vi "VirtualATE_V2_after_step8.vi"() -> ()   [LabVIEW 2026]
uses:
  <vilib>/NI/Modbus Library/API/Modbus API.lvclass/Modbus API.ctl
  <vilib>/NI/Modbus Library/Transmission Data Unit/Transmission Data Unit.lvclass/Transmission Data Unit.ctl
  <vilib>/NI/Modbus Library/Transmission Data Unit/Write Unit ID.vi
  <vilib>/NI/Modbus Library/API/Read Transmission Data Unit.vi
  <vilib>/NI/Modbus Library/API/Write Transmission Data Unit.vi
  <vilib>/NI/Modbus Library/API/Master/Modbus Master.lvclass
  C:/Program Files (x86)/National Instruments/LabVIEW 2026/vi.lib/NI/Modbus Library/API/Modbus API.lvclass
  <vilib>/NI/Modbus Library/API/Wrapper/Create TCP Master.vi
  <vilib>/NI/Modbus Library/API/Wrapper/API Main.lvlib
panel:
  out "PLC_HB_TIMEOUT":bool
  out "PLC_HB_AGE_MS":u32
  out "PLC_LIVE_OK":bool
  out "STATE_ELAPSED_MS":u32
  out "처리 메시지":string
  out "ATE_READY":bool
  out "ACTIVE_RESULT":u16
  out "ACTIVE_ID":u16
  out "ATE_STATE":u16
  out "PLC_LIVE_COUNTER":u16
  out "PLC_ACCEPTED_ID":u16
  out "PLC_RX_RESPONSE_ID":u16
  out "PLC_RX_DONE":u16
  out "PLC_RX_RESULT":u16
  in  "검사 결과 선택":enum16{"PASS", "FAIL", "RETEST"}(ring)
  out "바깥 Tick Count(ms)":u32
  in  "ATE 읽기 정지":bool
  out "ALARM_CODE":u16
  out "SEQ_STATE":u16
  out "TEEST_RESULT_LATCH":u16
  out "ATE_DONE":u16
  out "ATE_RESPONSE_ID":u16
  out "ATE_RESULT":u16
  out "ATE_REQUEST_ID":u16
  out "ATE_REQUEST":u16
  out "마지막 Modbus 읽기 정상":bool
  out "수신 레지스터":u16[](array[numeric])
  out "error out":errorcluster
  in  "Unit ID":u8
  in  "Port":u16
  in  "Server IP":string
  # "R[3]"
  # "R[4]"
  # "R[5]"
  # "R[6]"
  # "R[7]"
  # "R[8]"
  # "R[9]"
  # "R[10]"
  # "R[11]"
  # "R[12]"
  # "0 ATE_LINK_TEST\n1 ATE_REQUEST\n2 ATE_REQUEST_ID\n3 ATE_RESULT\n4 ATE_RESPONSE_ID\n5 ATE_DONE\n6 TEST_RESULT_LATCH\n7 SEQ_STATE\n8 ALARM_CODE"
  # "R[13]"
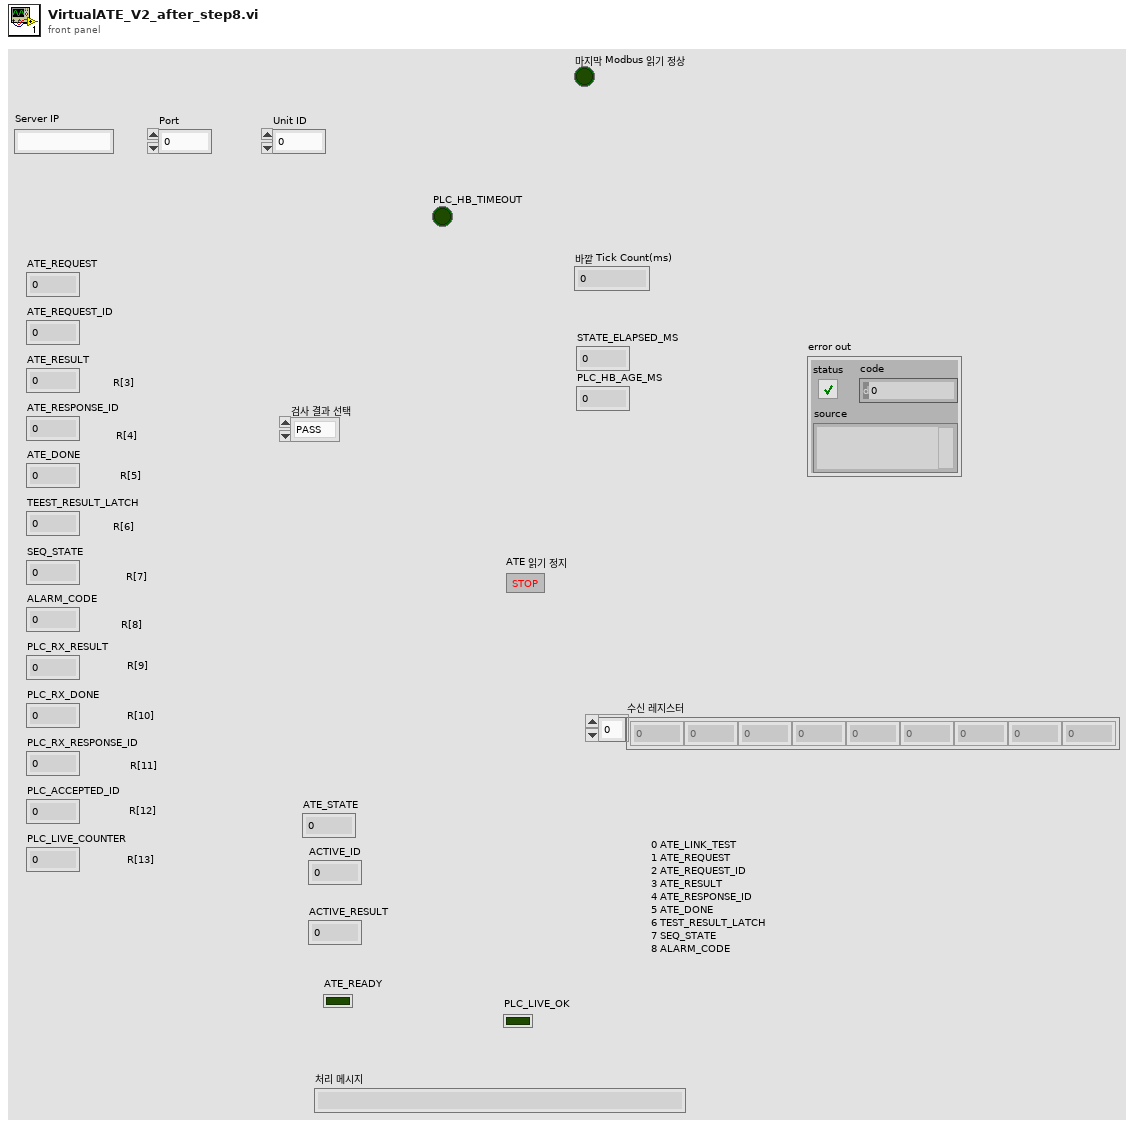
[diagram p1: front panel]
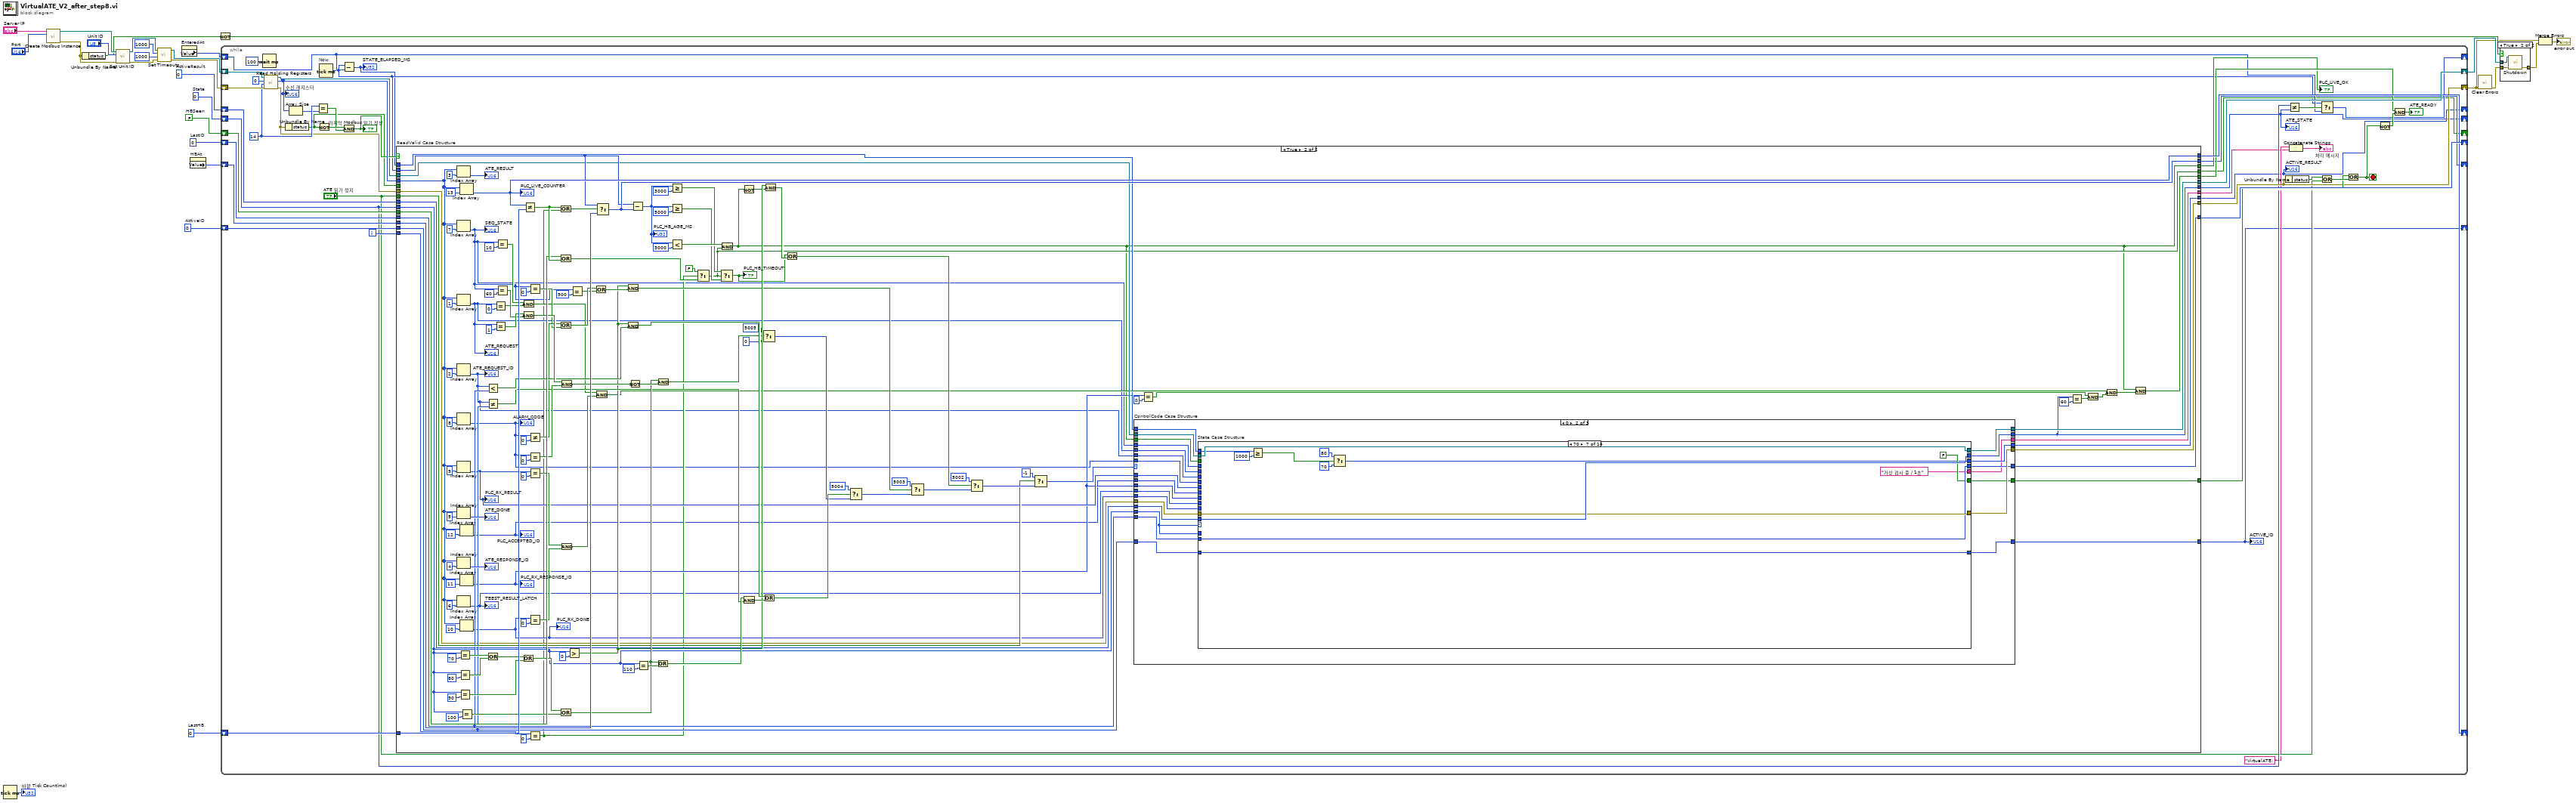
[diagram p0: block diagram]
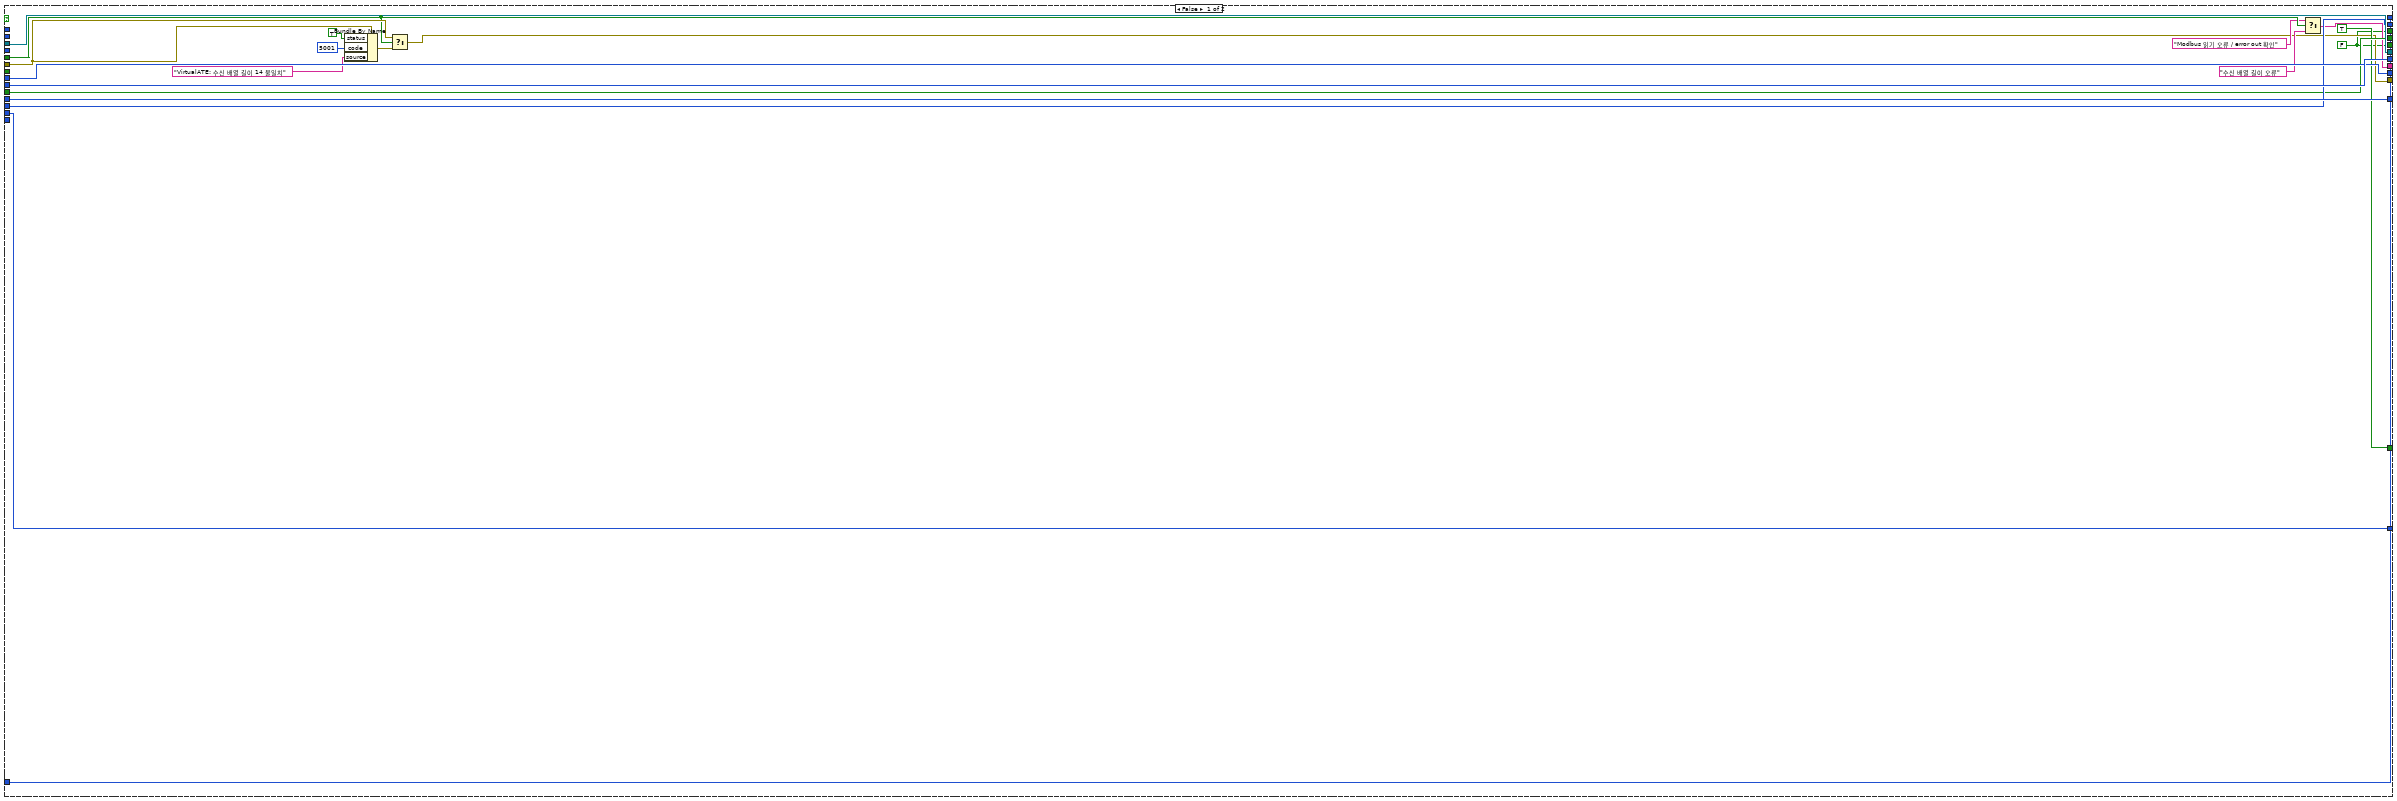
[diagram p3: hidden frame]
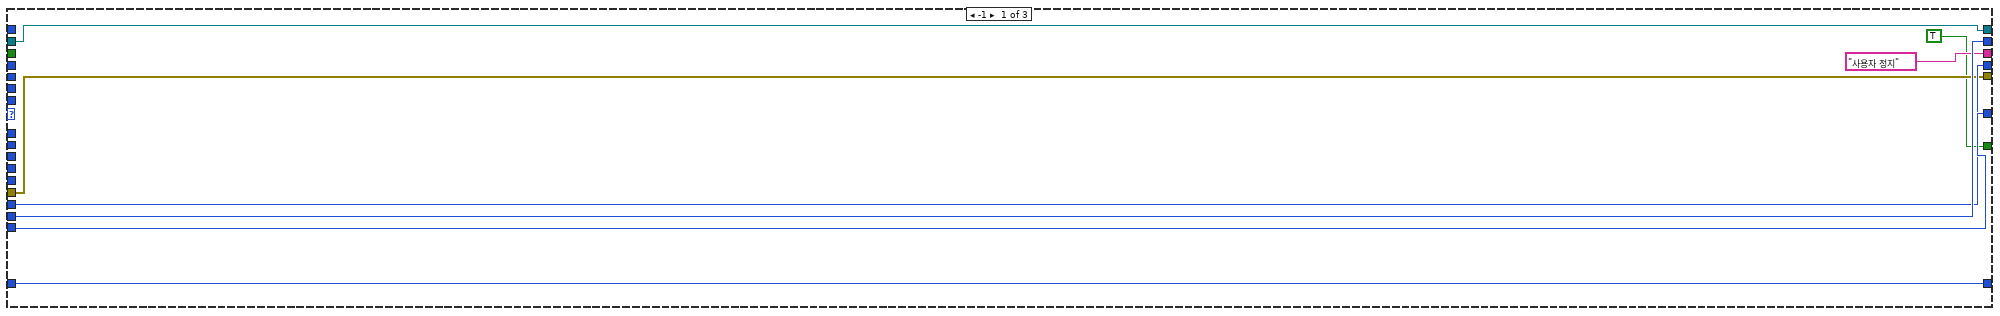
[diagram p4: hidden frame]
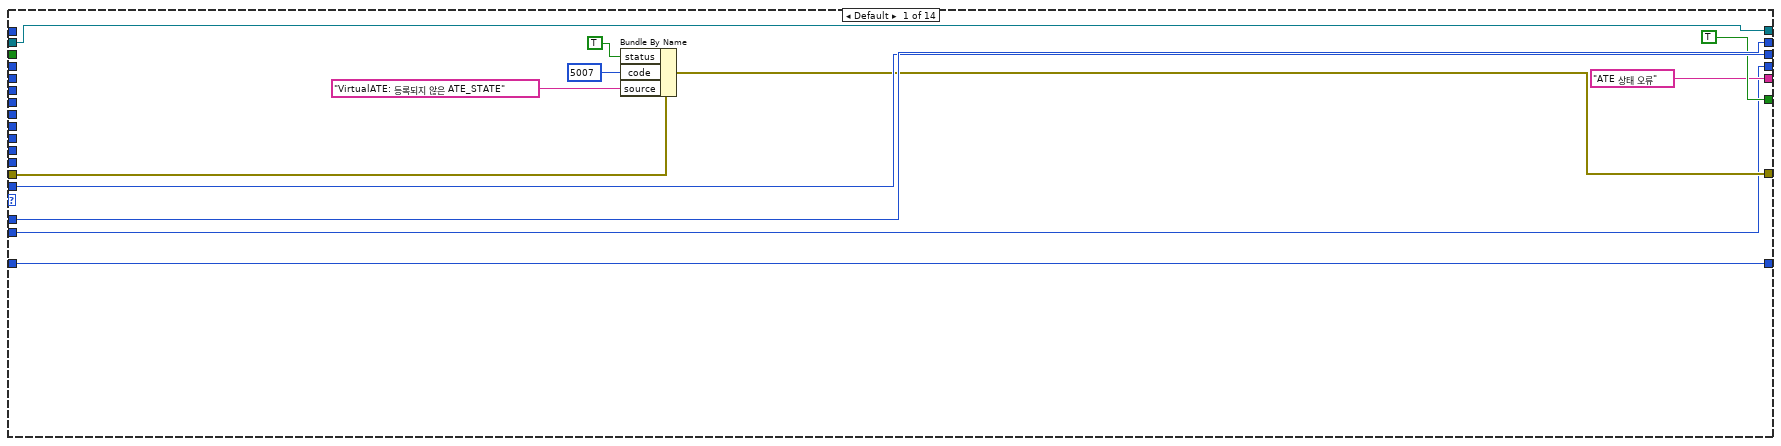
[diagram p5: hidden frame]
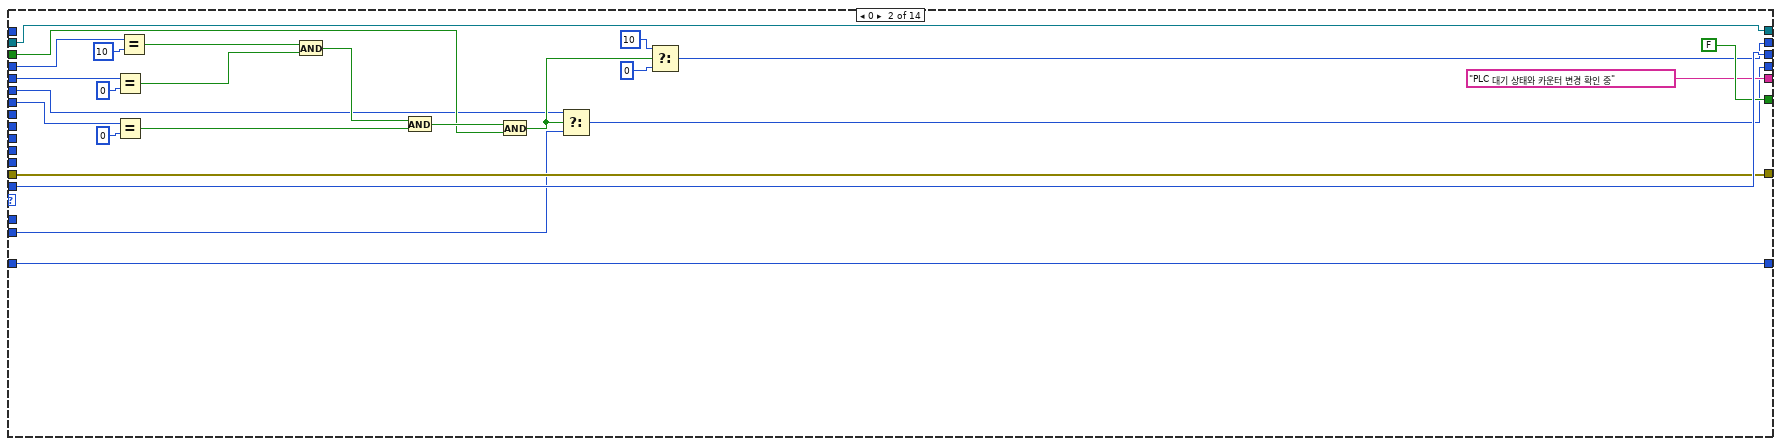
[diagram p6: hidden frame]
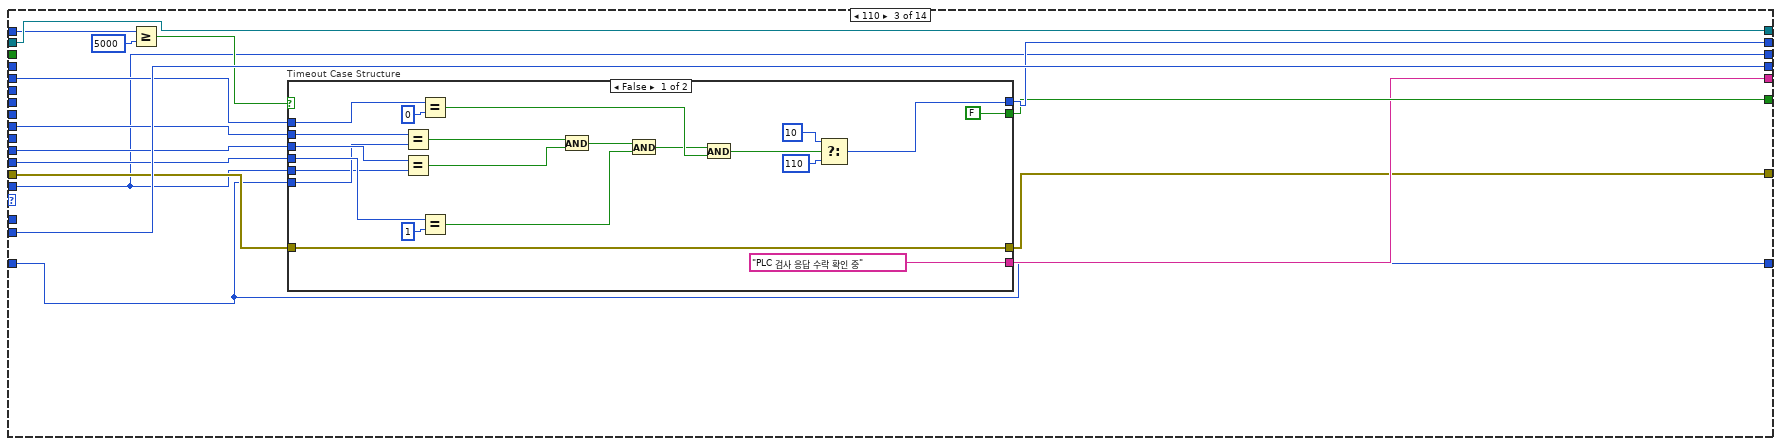
[diagram p7: hidden frame]
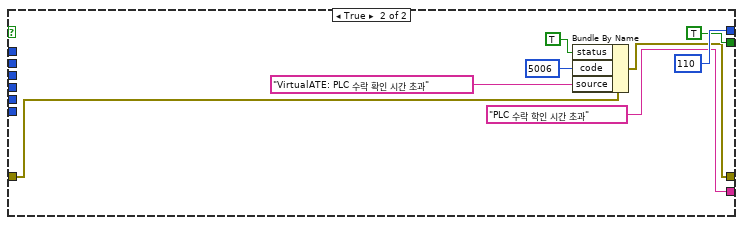
[diagram p8: hidden frame]
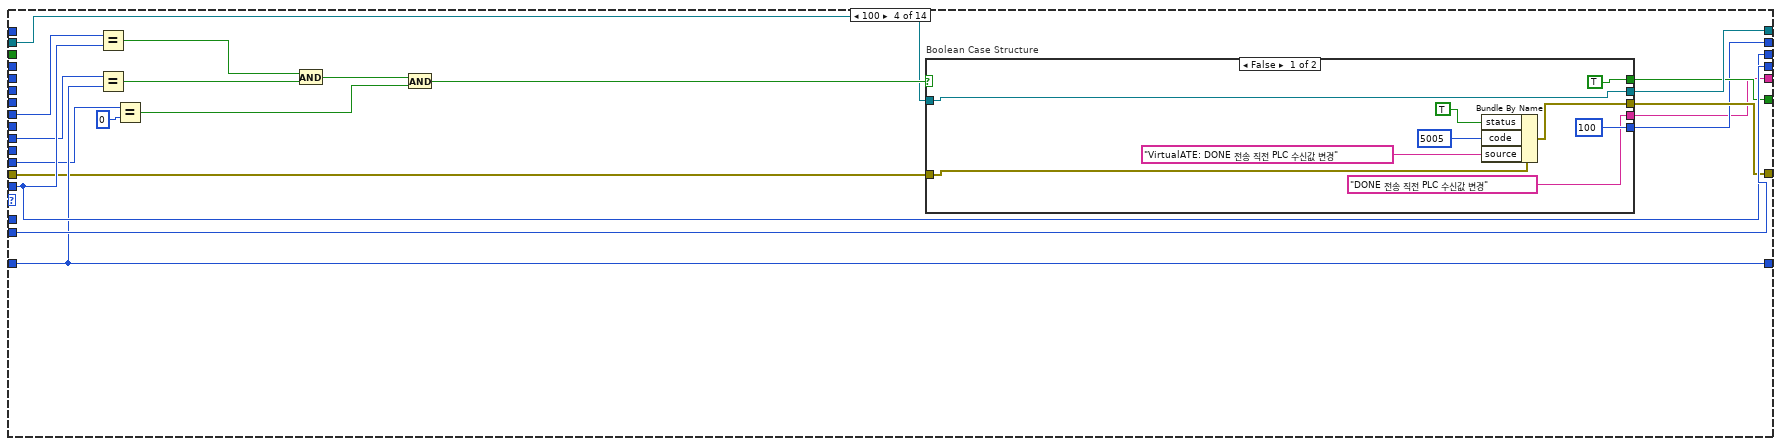
[diagram p9: hidden frame]
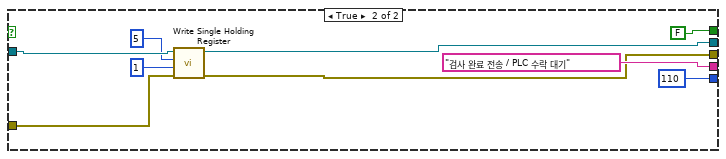
[diagram p10: hidden frame]
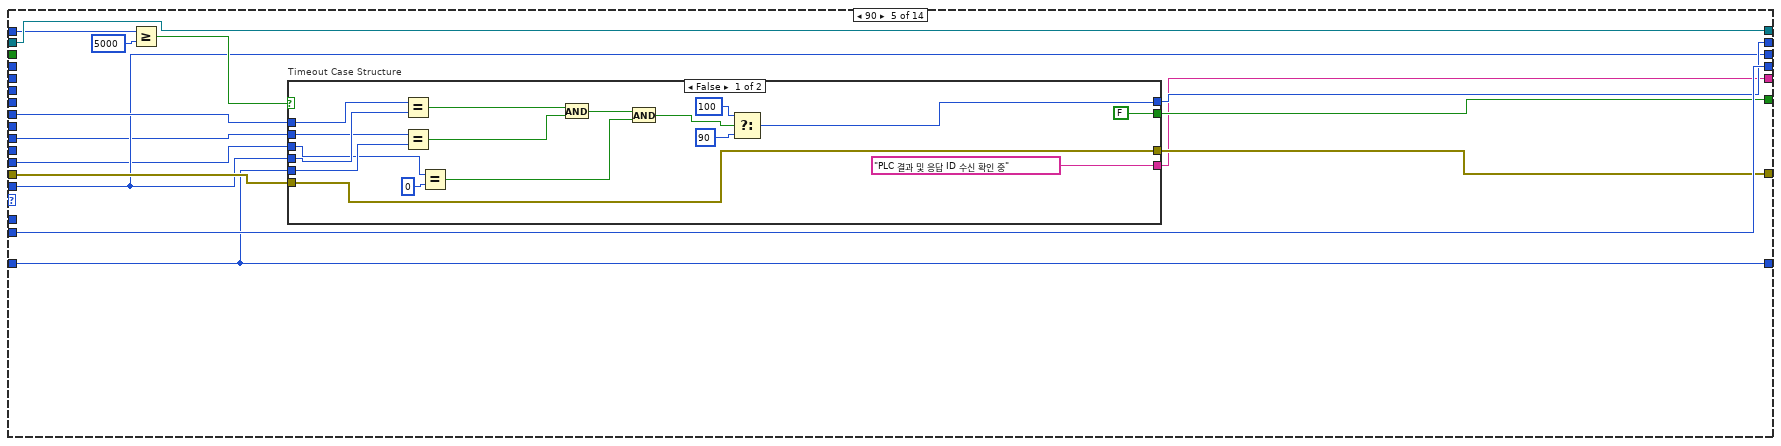
[diagram p11: hidden frame]
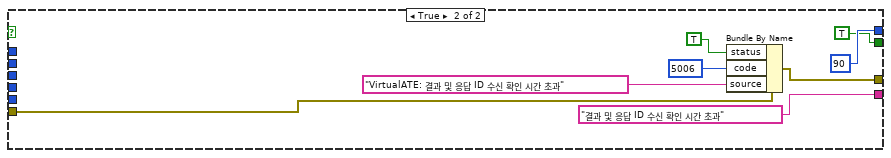
[diagram p12: hidden frame]
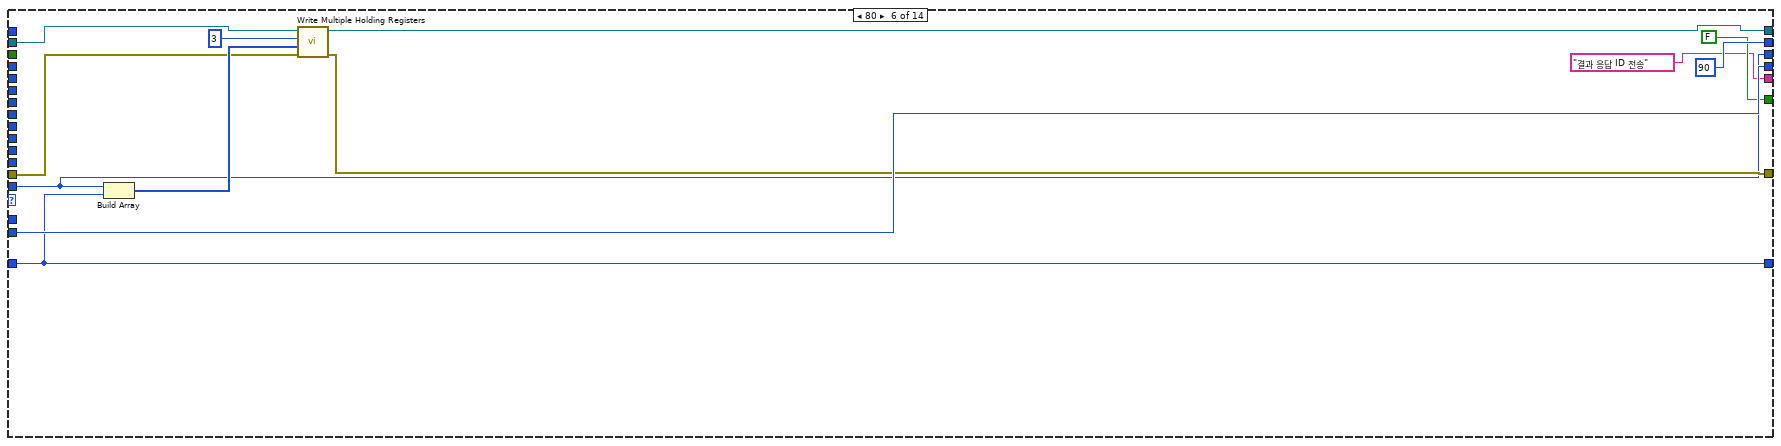
[diagram p13: hidden frame]
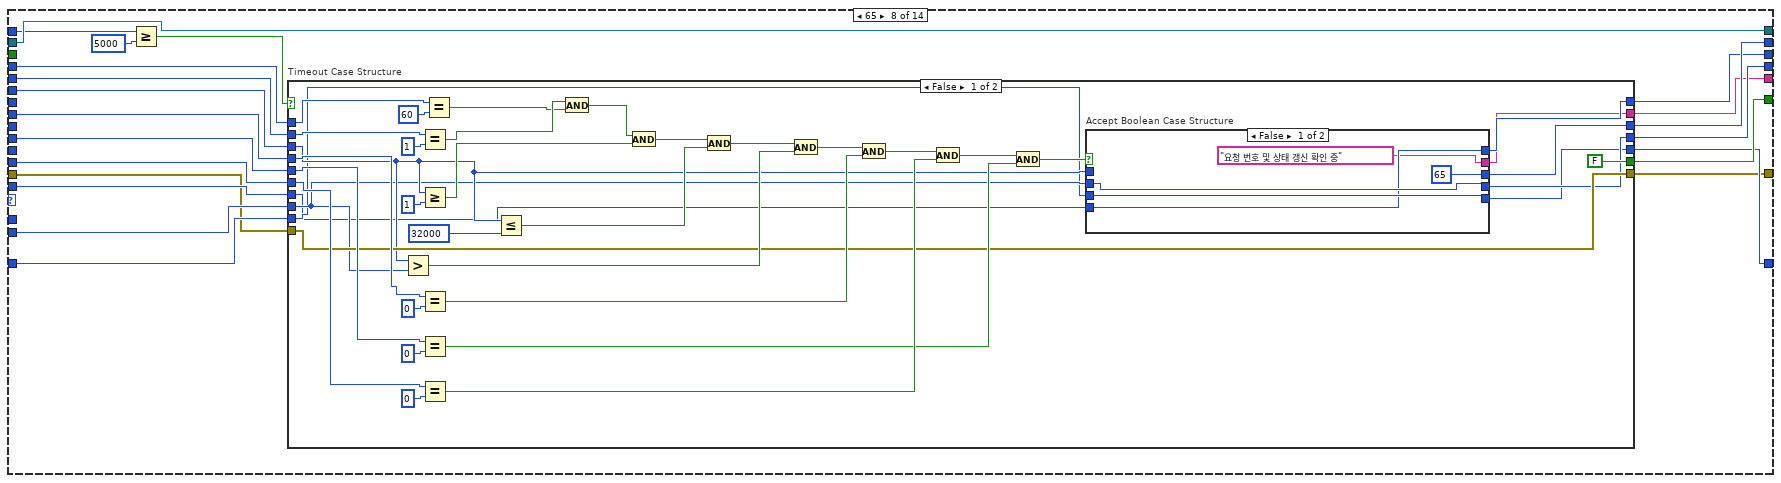
[diagram p14: hidden frame]
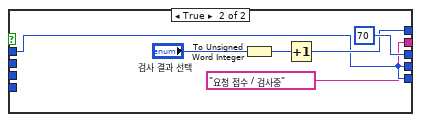
[diagram p15: hidden frame]
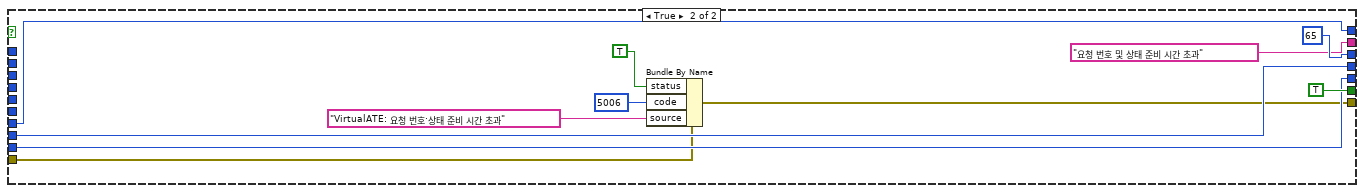
[diagram p16: hidden frame]
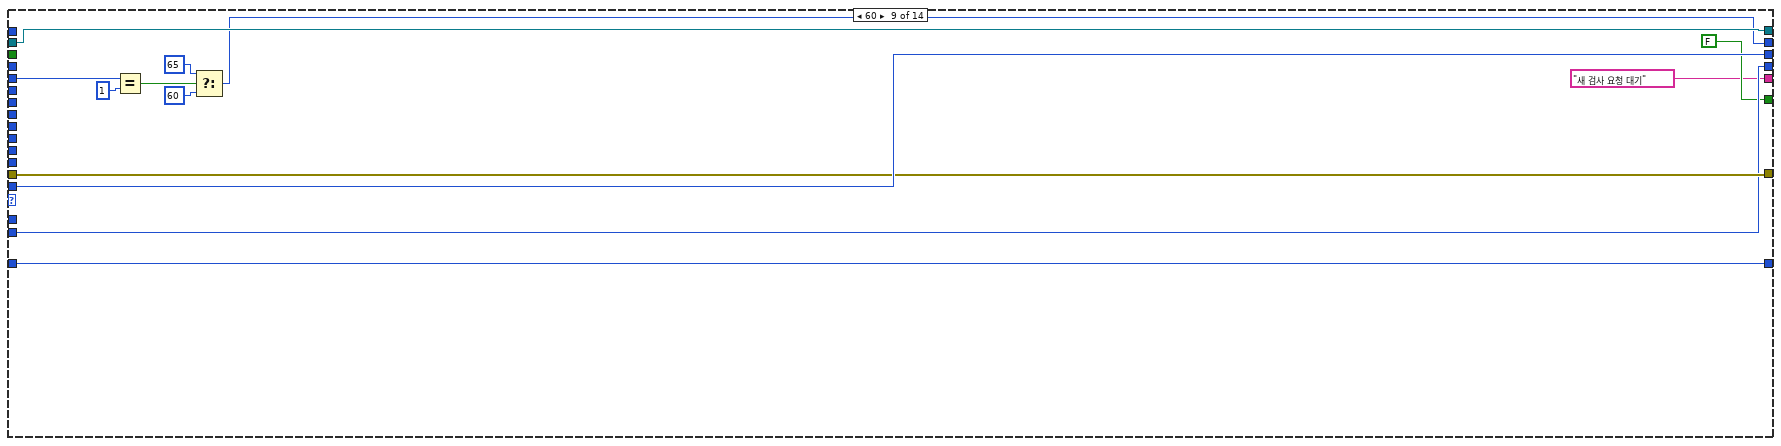
[diagram p17: hidden frame]
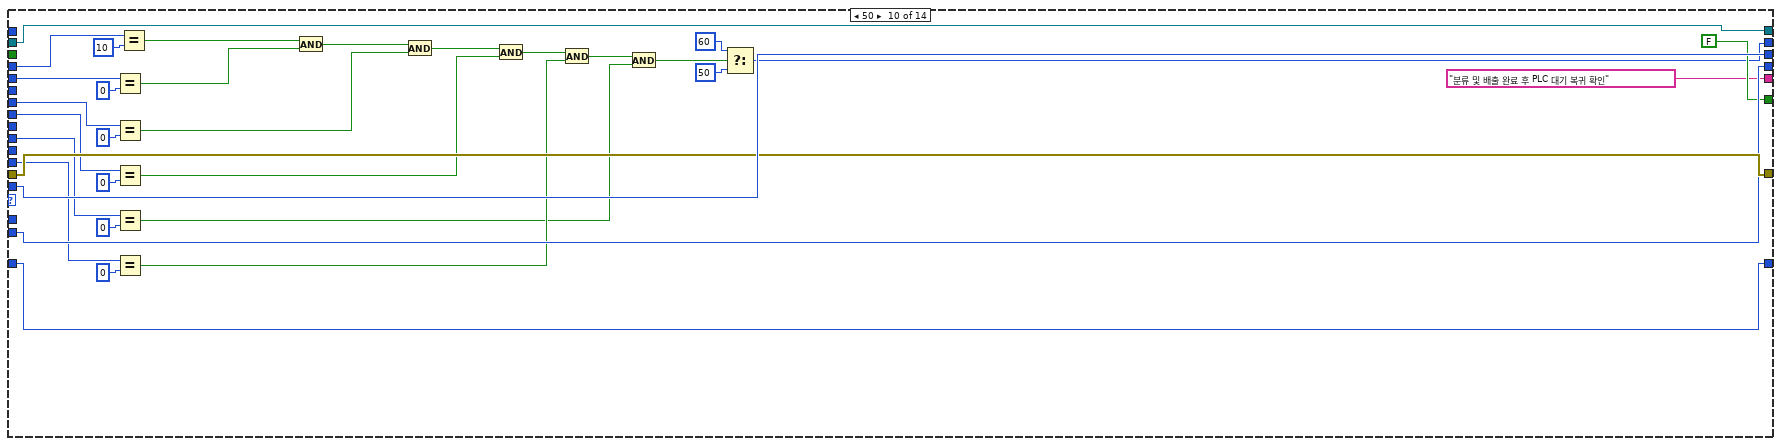
[diagram p18: hidden frame]
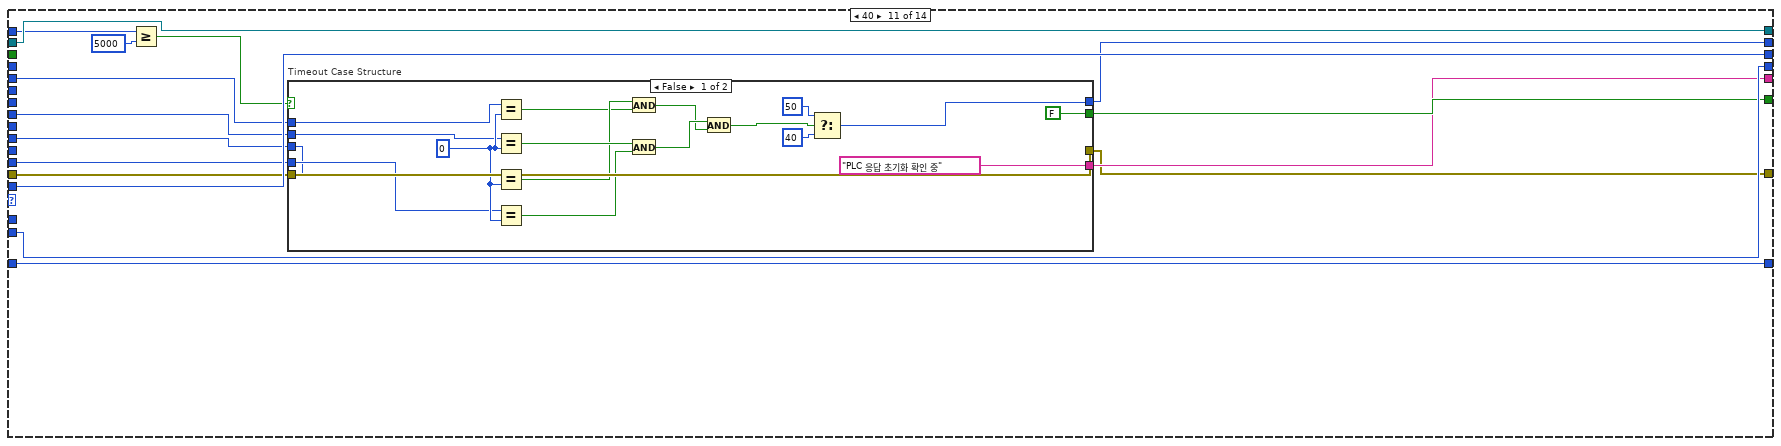
[diagram p19: hidden frame]
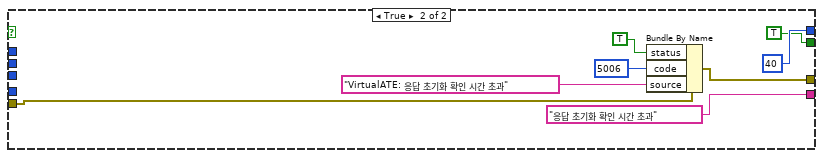
[diagram p20: hidden frame]
diagram:
  w9 = FALSE  # HBSeen
  w4 = u16 0  # LastHB
  w5 = u16 0  # ActiveResult
  w6 = u16 0  # ActiveID
  w7 = u16 0  # LastID
  w8 = u16 0  # State
  n1 = Tick Count (ms)() -> (millisecond timer value=→"바깥 Tick Count(ms)":u32)
  n2 = call-poly <vilib>:"Create Modbus Instance.vi"("port (502)"="Port", "address"="Server IP") -> ("error out"=w17:errorcluster, "TCP master instance"=w22:refnum<class "Modbus Master.lvclass">)  [unwired: 8 in]
  n3 = Unbundle By Name(w17) -> ("status"=w16:bool)
  n4 = call <vilib>:"Set Unit ID.vi"("error in"=w17, "unit ID"="Unit ID", "Modbus master in"=w22) -> ("error out"=w20:errorcluster, "Modbus master out"=w21:refnum<class "Modbus Master.lvclass">)  [unwired: 7 in]
  n5 = call <vilib>:"Set Timeouts.vi"("error in"=w20, "write operation timeout"=1000, "read operation timeout"=1000, "Modbus master in"=w21) -> ("error out"=w18:errorcluster, "Modbus master out"=w19:refnum<class "Modbus Master.lvclass">)  [unwired: 6 in]
  n6 = property on="EnteredAt" class="DigNum (strict)"() -> ("Value"=w2:u32)  [unwired: 2 in, 2 out]
  n7 = property on="HBAt" class="DigNum (strict)"() -> ("Value"=w1:u32)  [unwired: 2 in, 2 out]
  n8 = Not(x=w16) -> (.not. x?=w15:bool)
  n9 = while {
    shift-right: [w48] -> w11
    shift-left: w18 -> [w71]
    shift-right: [w59] -> w14
    shift-left: w19 -> [w72]
    shift-right: [w28] -> _
    shift-left: w8 -> [w40]
    shift-right: [w63] -> _
    shift-left: w7 -> [w64]
    shift-right: [w30] -> _
    shift-left: w6 -> [w62]
    shift-right: [w29] -> _
    shift-left: w5 -> [w61]
    shift-right: [w38] -> _
    shift-left: w1 -> [w55]
    shift-right: [w56] -> _
    shift-left: w4 -> [w57]
    shift-right: [w42] -> _
    shift-left: w2 -> [w39]
    shift-right: [w37] -> _
    shift-left: w9 -> [w54]
    i -> [w43]
    stop <- w45 stop-if-true
    w70 = u16 14 ("number of inputs")
    n10 = Wait (ms)(milliseconds to wait=u32 100) -> ()  [unwired: 1 out]
    n11 = call-dynamic "Read Holding Registers.vi"("error in"=w71, "number of inputs"=w70, "starting address"=u16 0, "Modbus master in"=w72) -> ("error out"=w58:errorcluster, "register values"=w66:u16[], "Modbus master out"=w60:refnum<class "Modbus Master.lvclass">)  [unwired: 5 in]
    "수신 레지스터" <- w66
    n12 = Unbundle By Name(w58) -> ("status"=w53:bool)
    n13 = Array Size(array=w66) -> (size(s)=w69:i32)
    n14 = Equal?(x=w70, y=w69) -> (x = y?=w67:bool)
    n15 = Not(x=w53) -> (.not. x?=w68:bool)
    n16 = Tick Count (ms) "Now"() -> (millisecond timer value=w36:u32)
    n17 = Subtract(x=w36, y=w39) -> (x-y=w34:u32)
    "STATE_ELAPSED_MS" <- w34
    n18 = And(x=w68, y=w67) -> (x .and. y?=w65:bool)
    "마지막 Modbus 읽기 정상" <- w65
    n19 = case "ReadValid Case Structure" shown="True" w65 {
      tunnel: w66 -> [_ w220]
      tunnel: w40 -> [w94 w127]
      tunnel: [w94 w121] -> w28
      tunnel: w64 -> [w93 w139]
      tunnel: [w93 w138] -> w63
      tunnel: w62 -> [w92 w137]
      tunnel: [w92 w136] -> w30
      tunnel: w61 -> [w91 w135]
      tunnel: [w91 w134] -> w29
      tunnel: w60 -> [w90 w133]
      tunnel: [w90 w132] -> w59
      tunnel: w58 -> [w82 w131]
      tunnel: [w76 w130] -> w48
      tunnel: w57 -> [w89 w212]
      tunnel: [w89 w209] -> w56
      tunnel: w55 -> [w88 w207]
      tunnel: [w88 w208] -> w38
      tunnel: w54 -> [w87 w210]
      tunnel: [w87 w102] -> w37
      tunnel: w53 -> [w80 _]
      tunnel: [TRUE w128] -> w51
      tunnel: [w77 w129] -> w32
      tunnel: [w75 w108] -> w49
      tunnel: [w75 w95] -> w44
      tunnel: w43 -> [_ w214]
      tunnel: w36 -> [_ w201]
      tunnel: "ATE 읽기 정지" -> [_ w141]
      tunnel: w34 -> [_ w107]
      frame False {
        w75 = FALSE
        n20 = Bundle By Name(cluster=w82, "status"=TRUE, "code"=5001, "source"="VirtualATE: 수신 배열 길이 14 불일치") -> (w83:errorcluster)
        n21 = Select(t=w82, s=w80, f=w83) -> (s? t:f=w76:errorcluster)
        n22 = Select(t="Modbus 읽기 오류 / error out 확인", s=w80, f="수신 배열 길이 오류") -> (s? t:f=w77:string)
      }
      frame True {
        n23 = Index Array(array=w220, index=3) -> (element=→"ATE_RESULT":u16)
        n24 = Index Array(array=w220, index=7) -> (element=w100:u16)
        "SEQ_STATE" <- w100
        n25 = Index Array(array=w220, index=1) -> (element=w103:u16)
        "ATE_REQUEST" <- w103
        n26 = Index Array(array=w220, index=2) -> (element=w98:u16)
        "ATE_REQUEST_ID" <- w98
        n27 = Index Array(array=w220, index=8) -> (element=w99:u16)
        "ALARM_CODE" <- w99
        n28 = Index Array(array=w220, index=9) -> (element=w105:u16)
        "PLC_RX_RESULT" <- w105
        n29 = Index Array(array=w220, index=5) -> (element=→"ATE_DONE":u16)
        n30 = Index Array(array=w220, index=4) -> (element=→"ATE_RESPONSE_ID":u16)
        n31 = Index Array(array=w220, index=6) -> (element=w96:u16)
        "TEEST_RESULT_LATCH" <- w96
        n32 = Equal?(x=w127, y=u16 70) -> (x = y?=w190:bool)
        n33 = Equal?(x=w127, y=u16 80) -> (x = y?=w189:bool)
        n34 = Equal?(x=w127, y=u16 90) -> (x = y?=w188:bool)
        n35 = Index Array(array=w220, index=13) -> (element=w209:u16)
        "PLC_LIVE_COUNTER" <- w209
        n36 = Index Array(array=w220, index=12) -> (element=w97:u16)
        "PLC_ACCEPTED_ID" <- w97
        n37 = Index Array(array=w220, index=11) -> (element=w104:u16)
        "PLC_RX_RESPONSE_ID" <- w104
        n38 = Index Array(array=w220, index=10) -> (element=w106:u16)
        "PLC_RX_DONE" <- w106
        n39 = Equal?(x=w127, y=u16 100) -> (x = y?=w186:bool)
        n40 = Less?(x=w98, y=w139) -> (x < y?=w172:bool)
        n41 = Not Equal?(x=w98, y=w137) -> (x != y?=w170:bool)
        n42 = Or(x=w190, y=w189) -> (x .or. y?=w187:bool)
        n43 = Equal?(x=w103, y=u16 0) -> (x = y?=w118:bool)
        n44 = Equal?(x=w103, y=u16 1) -> (x = y?=w179:bool)
        n45 = Equal?(x=w100, y=u16 10) -> (x = y?=w119:bool)
        n46 = Equal?(x=w100, y=u16 60) -> (x = y?=w178:bool)
        n47 = Or(x=w187, y=w188) -> (x .or. y?=w185:bool)
        n48 = And(x=w119, y=w118) -> (x .and. y?=w113:bool)
        n49 = And(x=w179, y=w178) -> (x .and. y?=w176:bool)
        n50 = Not Equal?(x=w209, y=w212) -> (x != y?=w211:bool)
        n51 = Equal?(x=w100, y=u16 0) -> (x = y?=w163:bool)
        n52 = Not Equal?(x=w99, y=u16 0) -> (x != y?=w164:bool)
        n53 = Equal?(x=w99, y=u16 0) -> (x = y?=w177:bool)
        n54 = Equal?(x=w105, y=u16 0) -> (x = y?=w117:bool)
        n55 = Equal?(x=w106, y=u16 0) -> (x = y?=w116:bool)
        n56 = Equal?(x=w214, y=0) -> (x = y?=w101:bool)
        n57 = Or(x=w211, y=w101) -> (x .or. y?=w205:bool)
        n58 = Or(x=w210, y=w211) -> (x .or. y?=w206:bool)
        n59 = Or(x=w164, y=w163) -> (x .or. y?=w162:bool)
        n60 = Or(x=w185, y=w186) -> (x .or. y?=w173:bool)
        n61 = And(x=w176, y=w177) -> (x .and. y?=w175:bool)
        n62 = And(x=w117, y=w116) -> (x .and. y?=w112:bool)
        n63 = Greater?(x=w127, y=u16 0) -> (0:w159:bool)
        n64 = Equal?(x=w100, y=u16 900) -> (x = y?=w161:bool)
        n65 = Or(x=w162, y=w161) -> (x .or. y?=w160:bool)
        n66 = And(x=w113, y=w112) -> (x .and. y?=w110:bool)
        n67 = Select(t=w201, s=w205, f=w207) -> (s? t:f=w208:u32)
        n68 = And(x=w159, y=w160) -> (x .and. y?=w151:bool)
        n69 = And(x=w159, y=w172) -> (x .and. y?=w169:bool)
        n70 = Not(x=w175) -> (.not. x?=w174:bool)
        n71 = Subtract(x=w201, y=w208) -> (x-y=w200:u32)
        "PLC_HB_AGE_MS" <- w200
        n72 = Equal?(x=w127, y=u16 110) -> (x = y?=w183:bool)
        n73 = Or(x=w173, y=w183) -> (x .or. y?=w171:bool)
        n74 = And(x=w173, y=w174) -> (x .and. y?=w155:bool)
        n75 = Greater Or Equal?(x=w200, y=u32 3000) -> (x >= y?=w197:bool)
        n76 = Greater Or Equal?(x=w200, y=u32 5000) -> (x >= y?=w196:bool)
        n77 = Less?(x=w200, y=u32 3000) -> (x < y?=w203:bool)
        n78 = Select(t=FALSE, s=w101, f=w206) -> (s? t:f=w102:bool)
        n79 = Select(t=w197, s=w102, f=w196) -> (s? t:f=w156:bool)
        "PLC_HB_TIMEOUT" <- w156
        n80 = And(x=w203, y=w102) -> (x .and. y?=w95:bool)
        n81 = Not(x=w95) -> (.not. x?=w158:bool)
        n82 = And(x=w171, y=w170) -> (x .and. y?=w168:bool)
        n83 = Select(t=5005, s=w155, f=0) -> (s? t:f=w148:i32)
        n84 = Or(x=w169, y=w168) -> (x .or. y?=w152:bool)
        n85 = And(x=w159, y=w158) -> (x .and. y?=w157:bool)
        n86 = Or(x=w156, y=w157) -> (x .or. y?=w150:bool)
        n87 = Select(t=5004, s=w152, f=w148) -> (s? t:f=w147:i32)
        n88 = Select(t=5003, s=w151, f=w147) -> (s? t:f=w145:i32)
        n89 = Select(t=5002, s=w150, f=w145) -> (s? t:f=w143:i32)
        n90 = Select(t=-1, s=w141, f=w143) -> (s? t:f=w140:i32)
        n91 = case "ControlCode Case Structure" shown="0" w140 {
          selector: w140 -> [_ _ w692]
          tunnel: w127 -> [w239 w247 w700]
          tunnel: [w239 w258 w700] -> w121
          tunnel: w139 -> [w238 w264 w699]
          tunnel: [w238 w255 w699] -> w138
          tunnel: w137 -> [w237 w263 w698]
          tunnel: [w237 w254 w698] -> w136
          tunnel: [w236 w260 w697] -> w134
          tunnel: w135 -> [w236 w262 w697]
          tunnel: [w235 w259 w696] -> w132
          tunnel: w133 -> [w235 w261 w696]
          tunnel: [w234 w257 w695] -> w130
          tunnel: w131 -> [w234 w256 w694]
          tunnel: ["사용자 정지" w252 w674] -> w129
          tunnel: [TRUE w253 TRUE] -> w128
          tunnel: w107 -> [_ w251 _]
          tunnel: w106 -> [_ w250 _]
          tunnel: w105 -> [_ w249 _]
          tunnel: w104 -> [_ w248 _]
          tunnel: w103 -> [_ w244 _]
          tunnel: w100 -> [_ w246 _]
          tunnel: w99 -> [_ w245 _]
          tunnel: w98 -> [_ w243 _]
          tunnel: w97 -> [_ w242 _]
          tunnel: w96 -> [_ w241 _]
          tunnel: w95 -> [_ w240 _]
          frame -1 {
          }
          frame 0 {
            n92 = case "State Case Structure" shown="70" w247 {
              tunnel: w264 -> [w265 w278 w316 w365 w397 w434 w445 w464 w539 w572 w589 w629 w642 w671]
              tunnel: w263 -> [w266 w298 w303 w361 w385 w424 w444 w460 w538 w571 w588 w628 w641 w670]
              tunnel: w262 -> [w275 w301 w302 w363 w387 w425 w448 w458 w542 w575 w591 w631 w644 w673]
              tunnel: w261 -> [w274 w300 w317 w351 w398 w428 w447 w469 w541 w574 w590 w625 w643 w667]
              tunnel: [w275 w301 w302 w363 w387 w425 w448 w457 w542 w575 w591 w631 w644 w673] -> w260
              tunnel: [w274 w300 w317 w350 w398 w426 w447 w469 w541 w574 w590 w623 w643 w666] -> w259
              tunnel: [w276 w280 w312 w348 w391 u16 90 w439 w465 w530 w545 w582 u16 40 w635 u16 20] -> w258
              tunnel: [w269 w299 w308 w352 w392 w427 w446 w455 w540 w573 w580 w622 w634 w665] -> w257
              tunnel: w256 -> [w273 w299 w309 w353 w393 w429 w446 w456 w540 w573 w581 w624 w633 w664]
              tunnel: [w265 w277 w316 w365 w397 w434 w445 w463 w539 w572 w589 w629 w642 w671] -> w255
              tunnel: [w266 w298 w303 w361 w385 w424 w444 w459 w538 w571 w588 w628 w641 w670] -> w254
              tunnel: [TRUE FALSE w311 w349 w390 FALSE FALSE w462 FALSE FALSE w584 FALSE w636 FALSE] -> w253
              tunnel: ["ATE 상태 오류" "PLC 대기 상태와 카운터 변경 확인 중" w310 w347 w389 "결과 응답 ID 전송" "가상 검사 중 / 1초" w461 "새 검사 요청 대기" "분류 및 배출 완료 후 PLC 대기 복귀 확인" w583 "결과 및 응답 ID 초기화 전송" w637 "DONE=0 전송 / PLC 반영 대기"] -> w252
              tunnel: w247 -> [w276 _ _ _ _ _ _ _ _ _ _ _ _ _]
              tunnel: w251 -> [_ _ w315 _ w396 _ w437 w467 _ _ w586 _ w639 _]
              tunnel: w250 -> [_ _ w305 w360 w384 _ _ w450 _ w564 w578 _ w632 _]
              tunnel: w249 -> [_ _ _ w364 w388 _ _ w451 _ w565 w579 _ _ _]
              tunnel: w248 -> [_ _ _ w362 w386 _ _ w449 _ w563 w577 _ _ _]
              tunnel: w244 -> [_ w293 w304 _ _ _ _ w454 w535 w567 w576 _ _ _]
              tunnel: w246 -> [_ w295 _ _ _ _ _ w453 _ w568 _ _ _ _]
              tunnel: w245 -> [_ w292 _ _ _ _ _ _ _ w566 _ _ _ _]
              tunnel: w243 -> [_ w279 _ _ _ _ _ w452 _ _ _ _ _ _]
              tunnel: w242 -> [_ _ w307 _ _ _ _ _ _ _ _ _ _ _]
              tunnel: w241 -> [_ _ w306 _ _ _ _ _ _ _ _ _ _ _]
              tunnel: w240 -> [_ w284 _ _ _ _ _ _ _ _ _ _ _ _]
              frame Default {
                n93 = Bundle By Name(cluster=w273, "status"=TRUE, "code"=5007, "source"="VirtualATE: 등록되지 않은 ATE_STATE") -> (w269:errorcluster)
              }
              frame 0 {
                n94 = Equal?(x=w293, y=u16 0) -> (x = y?=w288:bool)
                n95 = Equal?(x=w292, y=u16 0) -> (x = y?=w287:bool)
                n96 = Equal?(x=w295, y=u16 10) -> (x = y?=w289:bool)
                n97 = And(x=w289, y=w288) -> (x .and. y?=w286:bool)
                n98 = And(x=w286, y=w287) -> (x .and. y?=w285:bool)
                n99 = And(x=w285, y=w284) -> (x .and. y?=w283:bool)
                n100 = Select(t=w279, s=w283, f=w278) -> (s? t:f=w277:u16)
                n101 = Select(t=u16 10, s=w283, f=u16 0) -> (s? t:f=w280:u16)
              }
              frame 110 {
                n102 = Greater Or Equal?(x=w315, y=u32 5000) -> (x >= y?=w313:bool)
                n103 = case "Timeout Case Structure" shown="False" w313 {
                  tunnel: [w318 u16 110] -> w312
                  tunnel: [FALSE TRUE] -> w311
                  tunnel: ["PLC 검사 응답 수락 확인 중" "PLC 수락 학인 시간 초과"] -> w310
                  tunnel: w309 -> [w336 w343]
                  tunnel: [w336 w339] -> w308
                  tunnel: w307 -> [w335 _]
                  tunnel: w306 -> [w334 _]
                  tunnel: w305 -> [w333 _]
                  tunnel: w304 -> [w332 _]
                  tunnel: w303 -> [w331 _]
                  tunnel: w302 -> [w330 _]
                  frame False {
                    n104 = Equal?(x=w335, y=w331) -> (x = y?=w327:bool)
                    n105 = Equal?(x=w334, y=w330) -> (x = y?=w326:bool)
                    n106 = Equal?(x=w332, y=u16 0) -> (x = y?=w324:bool)
                    n107 = Equal?(x=w333, y=u16 1) -> (x = y?=w325:bool)
                    n108 = And(x=w327, y=w326) -> (x .and. y?=w323:bool)
                    n109 = And(x=w323, y=w325) -> (x .and. y?=w322:bool)
                    n110 = And(x=w322, y=w324) -> (x .and. y?=w321:bool)
                    n111 = Select(t=u16 10, s=w321, f=u16 110) -> (s? t:f=w318:u16)
                  }
                  frame True {
                    n112 = Bundle By Name(cluster=w343, "status"=TRUE, "code"=5006, "source"="VirtualATE: PLC 수락 확인 시간 초과") -> (w339:errorcluster)
                  }
                }
              }
              frame 100 {
                n113 = Equal?(x=w364, y=w363) -> (x = y?=w358:bool)
                n114 = Equal?(x=w362, y=w361) -> (x = y?=w357:bool)
                n115 = Equal?(x=w360, y=u16 0) -> (x = y?=w356:bool)
                n116 = And(x=w358, y=w357) -> (x .and. y?=w355:bool)
                n117 = And(x=w355, y=w356) -> (x .and. y?=w354:bool)
                n118 = case "Boolean Case Structure" shown="False" w354 {
                  tunnel: w353 -> [w370 w378]
                  tunnel: [w366 w377] -> w352
                  tunnel: w351 -> [w373 w380]
                  tunnel: [w373 w379] -> w350
                  tunnel: [TRUE FALSE] -> w349
                  tunnel: [u16 100 u16 110] -> w348
                  tunnel: ["DONE 전송 직전 PLC 수신값 변경" "검사 완료 전송 / PLC 수락 대기"] -> w347
                  frame False {
                    n119 = Bundle By Name(cluster=w370, "status"=TRUE, "code"=5005, "source"="VirtualATE: DONE 전송 직전 PLC 수신값 변경") -> (w366:errorcluster)
                  }
                  frame True {
                    n120 = call-dynamic "Write Single Holding Register.vi"("error in"=w378, "register to write"=u16 1, "address"=u16 5, "Modbus master in"=w380) -> ("error out"=w377:errorcluster, "Modbus master out"=w379:refnum<class "Modbus Master.lvclass">)  [unwired: 6 in]
                  }
                }
              }
              frame 90 {
                n121 = Greater Or Equal?(x=w396, y=u32 5000) -> (x >= y?=w394:bool)
                n122 = case "Timeout Case Structure" shown="False" w394 {
                  tunnel: w393 -> [w415 w423]
                  tunnel: [w415 w419] -> w392
                  tunnel: [w399 u16 90] -> w391
                  tunnel: [FALSE TRUE] -> w390
                  tunnel: ["PLC 결과 및 응답 ID 수신 확인 중" "결과 및 응답 ID 수신 확인 시간 초과"] -> w389
                  tunnel: w388 -> [w412 _]
                  tunnel: w387 -> [w411 _]
                  tunnel: w386 -> [w410 _]
                  tunnel: w385 -> [w409 _]
                  tunnel: w384 -> [w408 _]
                  frame False {
                    n123 = Equal?(x=w412, y=w411) -> (x = y?=w406:bool)
                    n124 = Equal?(x=w410, y=w409) -> (x = y?=w405:bool)
                    n125 = Equal?(x=w408, y=u16 0) -> (x = y?=w404:bool)
                    n126 = And(x=w406, y=w405) -> (x .and. y?=w403:bool)
                    n127 = And(x=w403, y=w404) -> (x .and. y?=w402:bool)
                    n128 = Select(t=u16 100, s=w402, f=u16 90) -> (s? t:f=w399:u16)
                  }
                  frame True {
                    n129 = Bundle By Name(cluster=w423, "status"=TRUE, "code"=5006, "source"="VirtualATE: 결과 및 응답 ID 수신 확인 시간 초과") -> (w419:errorcluster)
                  }
                }
              }
              frame 80 {
                n130 = Build Array(w425, w424) -> (w430:u16[])
                n131 = call-dynamic "Write Multiple Holding Registers.vi"("error in"=w429, "registers to write"=w430, "starting address"=u16 3, "Modbus master in"=w428) -> ("error out"=w427:errorcluster, "Modbus master out"=w426:refnum<class "Modbus Master.lvclass">)  [unwired: 6 in]
              }
              frame 70 {
                n132 = Greater Or Equal?(x=w437, y=u32 1000) -> (x >= y?=w438:bool)
                n133 = Select(t=u16 80, s=w438, f=u16 70) -> (s? t:f=w439:u16)
              }
              frame 65 {
                n134 = Greater Or Equal?(x=w467, y=u32 5000) -> (x >= y?=w466:bool)
                n135 = case "Timeout Case Structure" shown="False" w466 {
                  tunnel: [w478 u16 65] -> w465
                  tunnel: w464 -> [w472 w528]
                  tunnel: [w475 w528] -> w463
                  tunnel: [FALSE TRUE] -> w462
                  tunnel: [w473 "요청 번호 및 상태 준비 시간 초과"] -> w461
                  tunnel: w460 -> [w471 w525]
                  tunnel: [w474 w525] -> w459
                  tunnel: w458 -> [w470 w524]
                  tunnel: [w476 w524] -> w457
                  tunnel: w456 -> [w479 w523]
                  tunnel: [w479 w519] -> w455
                  tunnel: w454 -> [w507 _]
                  tunnel: w453 -> [w505 _]
                  tunnel: w452 -> [w477 _]
                  tunnel: w451 -> [w493 _]
                  tunnel: w450 -> [w487 _]
                  tunnel: w449 -> [w484 _]
                  frame False {
                    n136 = Greater?(x=w477, y=w472) -> (0:w494:bool)
                    n137 = Equal?(x=w507, y=u16 1) -> (x = y?=w503:bool)
                    n138 = Greater Or Equal?(x=w477, y=u16 1) -> (x >= y?=w499:bool)
                    n139 = Equal?(x=w493, y=u16 0) -> (x = y?=w488:bool)
                    n140 = Equal?(x=w484, y=u16 0) -> (x = y?=w482:bool)
                    n141 = Equal?(x=w487, y=u16 0) -> (x = y?=w485:bool)
                    n142 = Equal?(x=w505, y=u16 60) -> (x = y?=w502:bool)
                    n143 = Less Or Equal?(x=w477, y=u16 32000) -> (x <= y?=w496:bool)
                    n144 = And(x=w503, y=w502) -> (x .and. y?=w500:bool)
                    n145 = And(x=w500, y=w499) -> (x .and. y?=w497:bool)
                    n146 = And(x=w497, y=w496) -> (x .and. y?=w495:bool)
                    n147 = And(x=w495, y=w494) -> (x .and. y?=w491:bool)
                    n148 = And(x=w491, y=w488) -> (x .and. y?=w490:bool)
                    n149 = And(x=w490, y=w485) -> (x .and. y?=w489:bool)
                    n150 = And(x=w489, y=w482) -> (x .and. y?=w481:bool)
                    n151 = case "Accept Boolean Case Structure" shown="False" w481 {
                      tunnel: [u16 65 u16 70] -> w478
                      tunnel: w477 -> [_ w514]
                      tunnel: [w509 w515] -> w476
                      tunnel: [w511 w514] -> w475
                      tunnel: [w510 w514] -> w474
                      tunnel: ["요청 번호 및 상태 갱신 확인 중" "요청 접수 / 검사중"] -> w473
                      tunnel: w472 -> [w511 _]
                      tunnel: w471 -> [w510 _]
                      tunnel: w470 -> [w509 _]
                      frame False {
                      }
                      frame True {
                        n152 = To Unsigned Word Integer(number="검사 결과 선택") -> (unsigned 16bit integer=w517:u16)
                        n153 = Increment(x=w517) -> (x+1=w515:u16)
                      }
                    }
                  }
                  frame True {
                    n154 = Bundle By Name(cluster=w523, "status"=TRUE, "code"=5006, "source"="VirtualATE: 요청 번호·상태 준비 시간 초과") -> (w519:errorcluster)
                  }
                }
              }
              frame 60 {
                n155 = Equal?(x=w535, y=u16 1) -> (x = y?=w533:bool)
                n156 = Select(t=u16 65, s=w533, f=u16 60) -> (s? t:f=w530:u16)
              }
              frame 50 {
                n157 = Equal?(x=w567, y=u16 0) -> (x = y?=w555:bool)
                n158 = Equal?(x=w566, y=u16 0) -> (x = y?=w554:bool)
                n159 = Equal?(x=w565, y=u16 0) -> (x = y?=w552:bool)
                n160 = Equal?(x=w563, y=u16 0) -> (x = y?=w548:bool)
                n161 = Equal?(x=w564, y=u16 0) -> (x = y?=w550:bool)
                n162 = Equal?(x=w568, y=u16 10) -> (x = y?=w556:bool)
                n163 = And(x=w556, y=w555) -> (x .and. y?=w553:bool)
                n164 = And(x=w553, y=w554) -> (x .and. y?=w551:bool)
                n165 = And(x=w551, y=w552) -> (x .and. y?=w549:bool)
                n166 = And(x=w549, y=w550) -> (x .and. y?=w547:bool)
                n167 = And(x=w547, y=w548) -> (x .and. y?=w546:bool)
                n168 = Select(t=u16 60, s=w546, f=u16 50) -> (s? t:f=w545:u16)
              }
              frame 40 {
                n169 = Greater Or Equal?(x=w586, y=u32 5000) -> (x >= y?=w585:bool)
                n170 = case "Timeout Case Structure" shown="False" w585 {
                  tunnel: [FALSE TRUE] -> w584
                  tunnel: ["PLC 응답 초기화 확인 중" "응답 초기화 확인 시간 초과"] -> w583
                  tunnel: [w604 u16 40] -> w582
                  tunnel: w581 -> [w609 w614]
                  tunnel: [w609 w610] -> w580
                  tunnel: w579 -> [w602 _]
                  tunnel: w578 -> [w601 _]
                  tunnel: w577 -> [w600 _]
                  tunnel: w576 -> [w599 _]
                  frame False {
                    w603 = u16 0 ("y")
                    n171 = Equal?(x=w599, y=w603) -> (x = y?=w595:bool)
                    n172 = Equal?(x=w602, y=w603) -> (x = y?=w598:bool)
                    n173 = Equal?(x=w600, y=w603) -> (x = y?=w596:bool)
                    n174 = Equal?(x=w601, y=w603) -> (x = y?=w597:bool)
                    n175 = And(x=w596, y=w595) -> (x .and. y?=w593:bool)
                    n176 = And(x=w598, y=w597) -> (x .and. y?=w594:bool)
                    n177 = And(x=w594, y=w593) -> (x .and. y?=w592:bool)
                    n178 = Select(t=u16 50, s=w592, f=u16 40) -> (s? t:f=w604:u16)
                  }
                  frame True {
                    n179 = Bundle By Name(cluster=w614, "status"=TRUE, "code"=5006, "source"="VirtualATE: 응답 초기화 확인 시간 초과") -> (w610:errorcluster)
                  }
                }
              }
              frame 30 {
                n180 = Build Array(u16 0 ("element"), u16 0 ("element")) -> (w618:u16[])
                n181 = call-dynamic "Write Multiple Holding Registers.vi"("error in"=w624, "registers to write"=w618, "starting address"=u16 3, "Modbus master in"=w625) -> ("error out"=w622:errorcluster, "Modbus master out"=w623:refnum<class "Modbus Master.lvclass">)  [unwired: 6 in]
              }
              frame 20 {
                n182 = Greater Or Equal?(x=w639, y=u32 5000) -> (x >= y?=w638:bool)
                n183 = case shown="False" w638 {
                  tunnel: ["PLC DONE=0 확인 중" "DONE=0 수신 확인 시간 초과"] -> w637
                  tunnel: [FALSE TRUE] -> w636
                  tunnel: [w650 u16 20] -> w635
                  tunnel: [w651 w654] -> w634
                  tunnel: w633 -> [w651 w658]
                  tunnel: w632 -> [w645 _]
                  frame False {
                    n184 = Equal?(x=w645, y=u16 0) -> (x = y?=w647:bool)
                    n185 = Select(t=u16 30, s=w647, f=u16 20) -> (s? t:f=w650:u16)
                  }
                  frame True {
                    n186 = Bundle By Name(cluster=w658, "status"=TRUE, "code"=5006, "source"="VirtualATE: DONE=0 수신 확인 시간 초과") -> (w654:errorcluster)
                  }
                }
              }
              frame 10 {
                n187 = call-dynamic "Write Single Holding Register.vi"("error in"=w664, "register to write"=u16 0, "address"=u16 5, "Modbus master in"=w667) -> ("error out"=w665:errorcluster, "Modbus master out"=w666:refnum<class "Modbus Master.lvclass">)  [unwired: 6 in]
              }
            }
          }
          frame Default {
            n188 = Equal?(x=w692, y=5002) -> (x = y?=w682:bool)
            n189 = Equal?(x=w692, y=5003) -> (x = y?=w683:bool)
            n190 = Equal?(x=w692, y=5004) -> (x = y?=w684:bool)
            n191 = Equal?(x=w692, y=5005) -> (x = y?=w687:bool)
            n192 = Select(t="검사 요청 철회", s=w687, f="ATE 제어 고장" ("t")) -> (s? t:f=w678:string)
            n193 = Select(t="요청 번호 감소 또는 검사 중 변경", s=w684, f=w678) -> (s? t:f=w677:string)
            n194 = Select(t="PLC 알람 또는 운전 불가", s=w683, f=w677) -> (s? t:f=w676:string)
            n195 = Select(t="PLC 카운터 변경 중단", s=w682, f=w676) -> (s? t:f=w674:string)
            n196 = Bundle By Name(cluster=w694, "status"=TRUE, "code"=w692, "source"=w674) -> (w695:errorcluster)
          }
        }
        n197 = Equal?(x=w104, y=u16 0) -> (x = y?=w115:bool)
        n198 = Equal?(x=w121, y=u16 60) -> (x = y?=w114:bool)
        n199 = And(x=w115, y=w114) -> (x .and. y?=w111:bool)
        n200 = And(x=w110, y=w111) -> (x .and. y?=w109:bool)
        n201 = And(x=w95, y=w109) -> (x .and. y?=w108:bool)
      }
    }
    "PLC_LIVE_OK" <- w44
    "ATE_STATE" <- w28
    "ACTIVE_ID" <- w30
    "ACTIVE_RESULT" <- w29
    n202 = Unbundle By Name(w48) -> ("status"=w47:bool)
    n203 = Not Equal?(x=w40, y=w28) -> (x != y?=w41:bool)
    n204 = Concatenate Strings("VirtualATE: ", w32) -> (→"처리 메시지":string)
    n205 = Or(x=w47, y="ATE 읽기 정지") -> (x .or. y?=w52:bool)
    n206 = Select(t=w36, s=w41, f=w39) -> (s? t:f=w42:u32)
    n207 = Or(x=w51, y=w52) -> (x .or. y?=w45:bool)
    n208 = Not(x=w45) -> (.not. x?=w46:bool)
    n209 = And(x=w49, y=w46) -> (x .and. y?=→"ATE_READY":bool)
  }
  n210 = call <vilib>:"Clear Errors.vi"("error in (no error)"=w11) -> ("error out"=w10:errorcluster)  [unwired: 5 in, 1 out]
  n211 = case shown="True" w15 {
    tunnel: w14 -> [_ w704]
    tunnel: [w701 w703] -> w13
    tunnel: w10 -> [w701 w702]
    frame False {
    }
    frame True {
      n212 = call-dynamic "Shutdown.vi"("error in"=w702, "Modbus master in"=w704) -> ("error out"=w703:errorcluster)  [unwired: 9 in]
    }
  }
  n213 = Merge Errors(w11, w13) -> (→"error out":errorcluster)
